vi "UE_Ms_To_Seconds.vi"(1 "milliseconds":dbl) -> (0 "seconds":dbl)   [LabVIEW 2026]
doc: "INTENT: Convert milliseconds to seconds. INPUTS: milliseconds (double). OUTPUTS: seconds (double). DESIGN CONSTRAINT: REQUIREMENTS: SRS-F-006. No physical hardware side effects. Acceptance requires native LabVIEW compilation and behavioral testing."
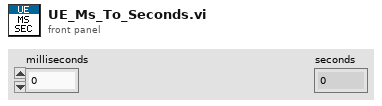
[diagram p1: front panel]
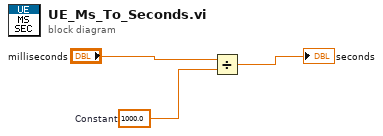
[diagram p0: block diagram]
diagram:
  w2 = 1000.0  # Constant
  n1 = Divide(x="milliseconds", y=w2) -> (x/y=→"seconds":dbl)
